vi "regexINI.vi"(8 "error in":errorcluster, 10 "INI String":string="[sectionName]\ntext = \"string\"\ncode = 123 // comment\n;code = 124\n\n[sectionName2]\ntext = \"string2\"\ncode = 345\n") -> (0 "error out":errorcluster, 2 "Sections":cluster{"section":string, "content":string}[](array[cluster]))   [LabVIEW 2013, in "CfgManager.Text.lvlib" / "ConfigManager.Text.INI.lvclass"]
uses:
  ConfigManager.Text.INI.lvclass
  <vilib>/LabVIEW Open Source Project/Serializer/Serializer.INI/Serializer.PlainText.INI.lvclass
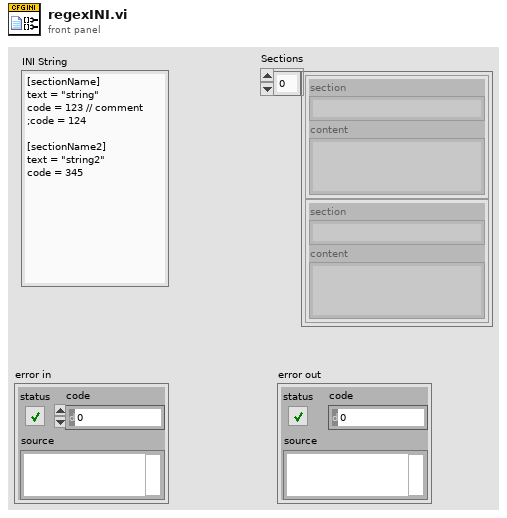
[diagram p1: front panel]
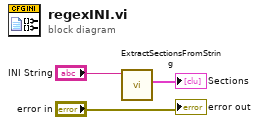
[diagram p0: block diagram]
diagram:
  n1 = call <vilib>:"ExtractSectionsFromString.vi"("String"="INI String") -> ("Sections"=→"Sections":cluster{"key":string, "value":string}[])  [unwired: 9 in, 1 out]
  "error out" <- "error in"
